vi "Parse Set TDF File.vi"(8 "error in (no error)":errorcluster caption="에러 입력(에러 없음)", 10 "JSON string":string, 11 "Instrument Manager 입력":refnum<class "Instrument Manager.lvclass">) -> (0 "error out":errorcluster caption="에러 출력", 1 "TDF File Name":string, 2 "Set TDF File Param":T1, 3 "Instrument Manager 출력":refnum<class "Instrument Manager.lvclass">)   [LabVIEW 2023, in "Instrument Manager.lvclass"]
uses:
  Instrument Manager.lvclass
  Instrument Manager.lvclass/Instrument Manager.ctl
  Set TDF File Param.ctl
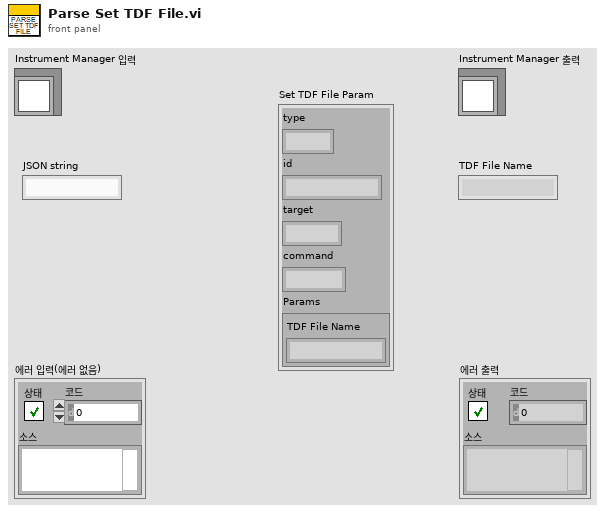
[diagram p1: front panel]
types:
  T1 = typedef "Instrument Manager.lvclass/Set TDF File Param.ctl" = cluster{"type":string, "id":string, "target":string, "command":string, "Params":cluster{"TDF File Name":string}}
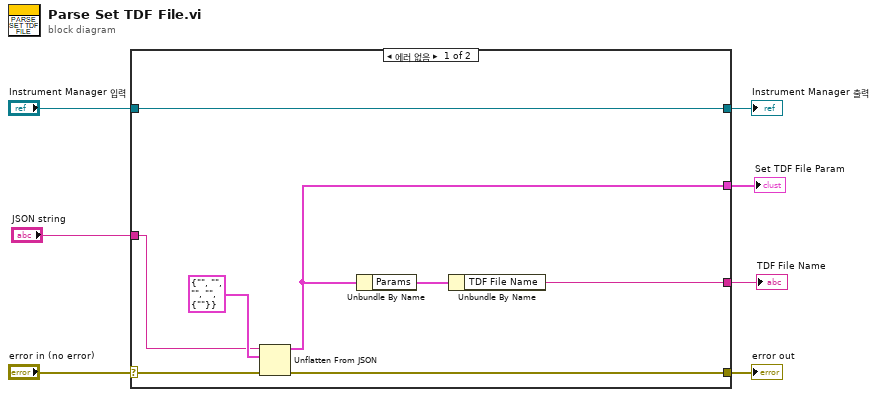
[diagram p0: block diagram]
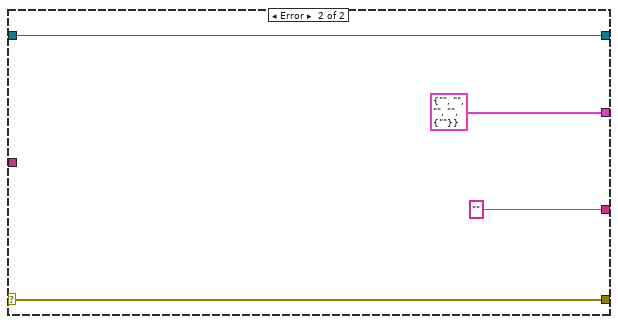
[diagram p2: hidden frame]
diagram:
  n1 = case shown="에러 없음" "error in (no error)" {
    selector: "error in (no error)" -> [w14 w19]
    tunnel: [w11 w19] -> w6
    tunnel: [w15 w18] -> w4
    tunnel: "Instrument Manager 입력" -> [w15 w18]
    tunnel: "JSON string" -> [w12 _]
    tunnel: [w9 T1 {"type"="", "id"="", "target"="", "command"="", "Params"={"TDF File Name"=""}} ("Set TDF File Param")] -> w2
    tunnel: [w8 "" ("TDF File Name")] -> w1
    frame No Error {
      n2 = Unflatten From JSON(JSON string=w12, type and defaults=T1 {"type"="", "id"="", "target"="", "command"="", "Params"={"TDF File Name"=""}} ("Set TDF File Param"), error in (no error)=w14) -> (value=w9:T1, error out=w11:errorcluster)  [unwired: 4 in]
      n3 = Unbundle By Name(w9) -> ("Params"=w10:cluster{"TDF File Name":string})
      n4 = Unbundle By Name(w10) -> ("TDF File Name"=w8:string)
    }
    frame Error {
    }
  }
  "error out" <- w6
  "Instrument Manager 출력" <- w4
  "Set TDF File Param" <- w2
  "TDF File Name" <- w1
